vi "Knock Sensor.vi"() -> ()   [LabVIEW 2016]
doc: "This example demonstrates how to acquire a single buffer of voltage measurements using a DAQmx device.\n\nFor instructions on how to connect your signals to the DAQ device, refer to your device documentation."
uses:
  <vilib>/Utility/error.llb/DialogType.ctl
  <vilib>/DAQmx/read.llb/DAQmx Read (Analog Wfm 1Chan NSamp Duration).vi
  <vilib>/addons/_NISVFA/_Spectrum Processing/SVFA Unit Conversion (1 Ch).vi
  <vilib>/addons/_NISVFA/_Spectrum Processing/SVFA Power in Band (1 Ch).vi
  <vilib>/addons/_NISVFA/_Shared subVIs/Common/svc_Spectrum Units.vi
  <vilib>/addons/_NISVFA/_Spectrum Processing/subVIs/svfa_Conversion Utility (spectrum info).vi
  <vilib>/addons/_NISVFA/_Spectrum Processing/SVFA Get Spectrum Subset.vi
  <vilib>/addons/_NISVFA/_Spectrum Processing/SVFA Get Spectrum Subset (1 Ch).vi
  <vilib>/addons/_NISVFA/_Spectrum Processing/subVIs/svfa_Peak to RMS to Peak2Peak.vi
  <vilib>/addons/_NISVFA/_Spectrum Processing/subVIs/svfa_Mag to Mag2.vi
  <vilib>/addons/_NISVFA/_Spectrum Processing/subVIs/svfa_Linear to dB.vi
  <vilib>/addons/_NISVFA/_Spectrum Processing/subVIs/svfa_dBrefA to dBrefB.vi
  <vilib>/addons/_NISVFA/_Spectrum Processing/subVIs/svfa_Spectrum to Spectral Density.vi
  <vilib>/DAQmx/create/channels.llb/DAQmx Create Channel (AI-Voltage-Basic).vi
  <vilib>/DAQmx/configure/timing.llb/DAQmx Timing (Sample Clock).vi
  <vilib>/DAQmx/miscellaneous.llb/DAQmx Fill In Error Info.vi
  <vilib>/addons/_NISVFA/_Baseband FFT/SVFA Power Spectrum (1 Ch).vi
  <vilib>/addons/_NISVFA/_Shared subVIs/Common/svc_Format Value (DBL).vi
  <vilib>/addons/_NISVFA/_Shared subVIs/Common/svc_Engineering Units to Unit Label.vi
  <vilib>/addons/_NISVFA/_Shared subVIs/Common/svc_Unit Label Lexical Class.vi
  <vilib>/addons/_NISVFA/_Shared subVIs/Common/svc_Get Weighting Enum and Labels.vi
  <vilib>/addons/_NISVFA/_Shared subVIs/Common/svc_Window Parameters.vi
  <vilib>/addons/_NISVFA/_Shared subVIs/Common/svc_Caller VI Returned in Error Source.vi
  <vilib>/addons/_NISVFA/_Shared subVIs/Common/svc_Check Frequency Range in Spectrum.vi
  <vilib>/addons/_NISVFA/_Shared subVIs/Common/svc_Convert Frequency to Frequency String.vi
  <vilib>/addons/_NISVFA/_Shared subVIs/Common/svc_Build Unit Label for Frequency Range.vi
  <vilib>/addons/_NISVFA/_Spectrum Processing/subVIs/svfa_Spectrum Info Window to windowTd Type Def.vi
panel:
  out "All duration within tolerance":bool=TRUE
  out "Measured Knock Magnitude":dbl=5.233809983966037
  in  "RPM":dbl=6000.0
  out "Pass?":bool
  out "Measured Base Magnitude":dbl=0.1959823715521759
  out "Indice of Samples of Base Component":i32[](array[numeric])
  out "Indice of Samples of Knock Component":i32[](array[numeric])
  out "Extracted Base Spectrum":cluster{"x0":dbl, "dx":dbl, "magnitude":dbl[]}(graph)={"x0"=0.0, "dx"=0.2253587147341788, "magnitude"=array[221869 elements]}
  out "Extracted Knock Spectrum":cluster{"x0":dbl, "dx":dbl, "magnitude":dbl[]}(graph)={"x0"=0.0, "dx"=1.9895350456598349, "magnitude"=array[25132 elements]}
  out "Extracted Knock Waveform":waveform(dbl)(graph)={"t0"=timestamp(0 s since 1904-01-01), "dt"=9.999999999999972e-06, "Y"=array[50263 elements]}
  out "Extracted Base Waveform":waveform(dbl)(graph)={"t0"=timestamp(0 s since 1904-01-01), "dt"=9.999999999999972e-06, "Y"=array[443737 elements]}
  in  "Knock Duration":dbl=0.002
  in  "Knock Amplityde":dbl=5.0
  in  "Base Frequency":dbl=6500.0
  in  "Base Amplitude":dbl=0.2
  in  "Knock Frequency":dbl=2000.0
  in  "Moving Window Size(how much of one knock cycle)":dbl=0.5
  out "Waveform Graph":waveform(dbl)(graph)={"t0"=timestamp(3584720197.6212864 s since 1904-01-01), "dt"=9.999999999999972e-06, "Y"=array[500000 elements], "attributes"=variant("NI_ChannelName"=variant(string "cDAQ1Mod3/ai1"), "NI_UnitDescription"=variant(string "Volts"))}
  in  "Sampling Rate":dbl=100000.0
  in  "Duration":i32=5
  in  "Sample Clock Source":tag="OnboardClock"
  in  "Terminal Configuration":i32(ring)=-1 items=["default"=-1, "RSE"=10083, "NRSE"=10078, "Differential"=10106, "Pseudodifferential"=12529]
  in  "Max Voltage":dbl=10.0
  in  "Min Voltage":dbl=-10.0
  in  "Physical Channel":tag="cDAQ1Mod3/ai1"
  # "This test uses a moving window to separate base component and knock component from the raw signal\nand verifies the frquency and magnitude of these two components, and duration of each knock event."
  # "Channel Settings"
  # "Acquired Data"
  # "Timing Settings"
  # "Extracted Knock Component Waveform"
  # "Extracted Knock Component Spectrum"
  # "Signal Parameters"
  # "Extracted Base Component Waveform"
  # "Extracted Base Component Spectrum"
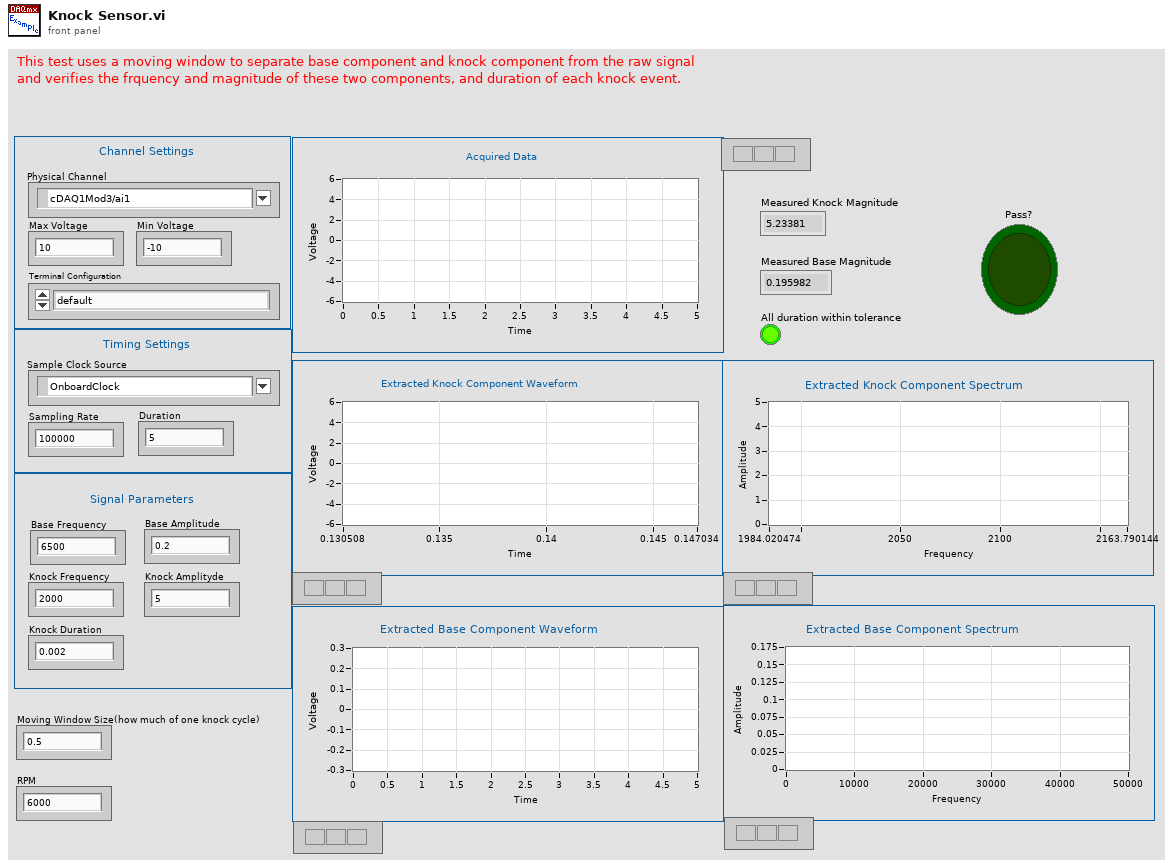
[diagram p1: front panel]
types:
  T1 = cluster{"linear/dB":enum16{"no change", "linear", "dB"}, "dB reference (0: no change)":dbl, "power/magnitude":enum16{"no change", "power", "magnitude"}, "view":enum16{"no change", "rms", "peak", "peak-peak"}}
  T2 = typedef "DialogType.ctl" = u16
  T3 = typedef "svc_Spectrum Info.ctl" = cluster{"channel name":string, "description":string, "x-axis units":T4, "spectral info":cluster{"spectrum type":T5, "linear/dB":enum16{"linear", "dB"}, "window":u16, "window size":i32, "FFT size":i32}, "engineering units":T6, "custom label":string, "dB reference [EU]":dbl, "peak units":enum16{"rms", "peak", "peak-peak"}, "weighting filter":T7, "spectral density?":bool, "unit label":string, "spectrum skewed?":bool, "complimentary spectrum units":T8}
  T4 = typedef "svc_X-Axis Units.ctl" = u16
  T5 = typedef "svc_Spectrum Type.ctl" = enum16{"FFT Spectrum [complex]", "Amplitude [Magnitude]", "Power [Magnitude^2]", "Cross Spectrum [complex]", "Frequency Response [Complex]"}
  T6 = typedef "svc_Engineering Units Text Ring.ctl" = u16
  T7 = typedef "svc_Weighting Filter Text Ring.ctl" = u16
  T8 = typedef "svc_Complimentary Spectrum Units.ctl" = enum16{"none", "radians", "degrees", "cycles", "imaginary"}
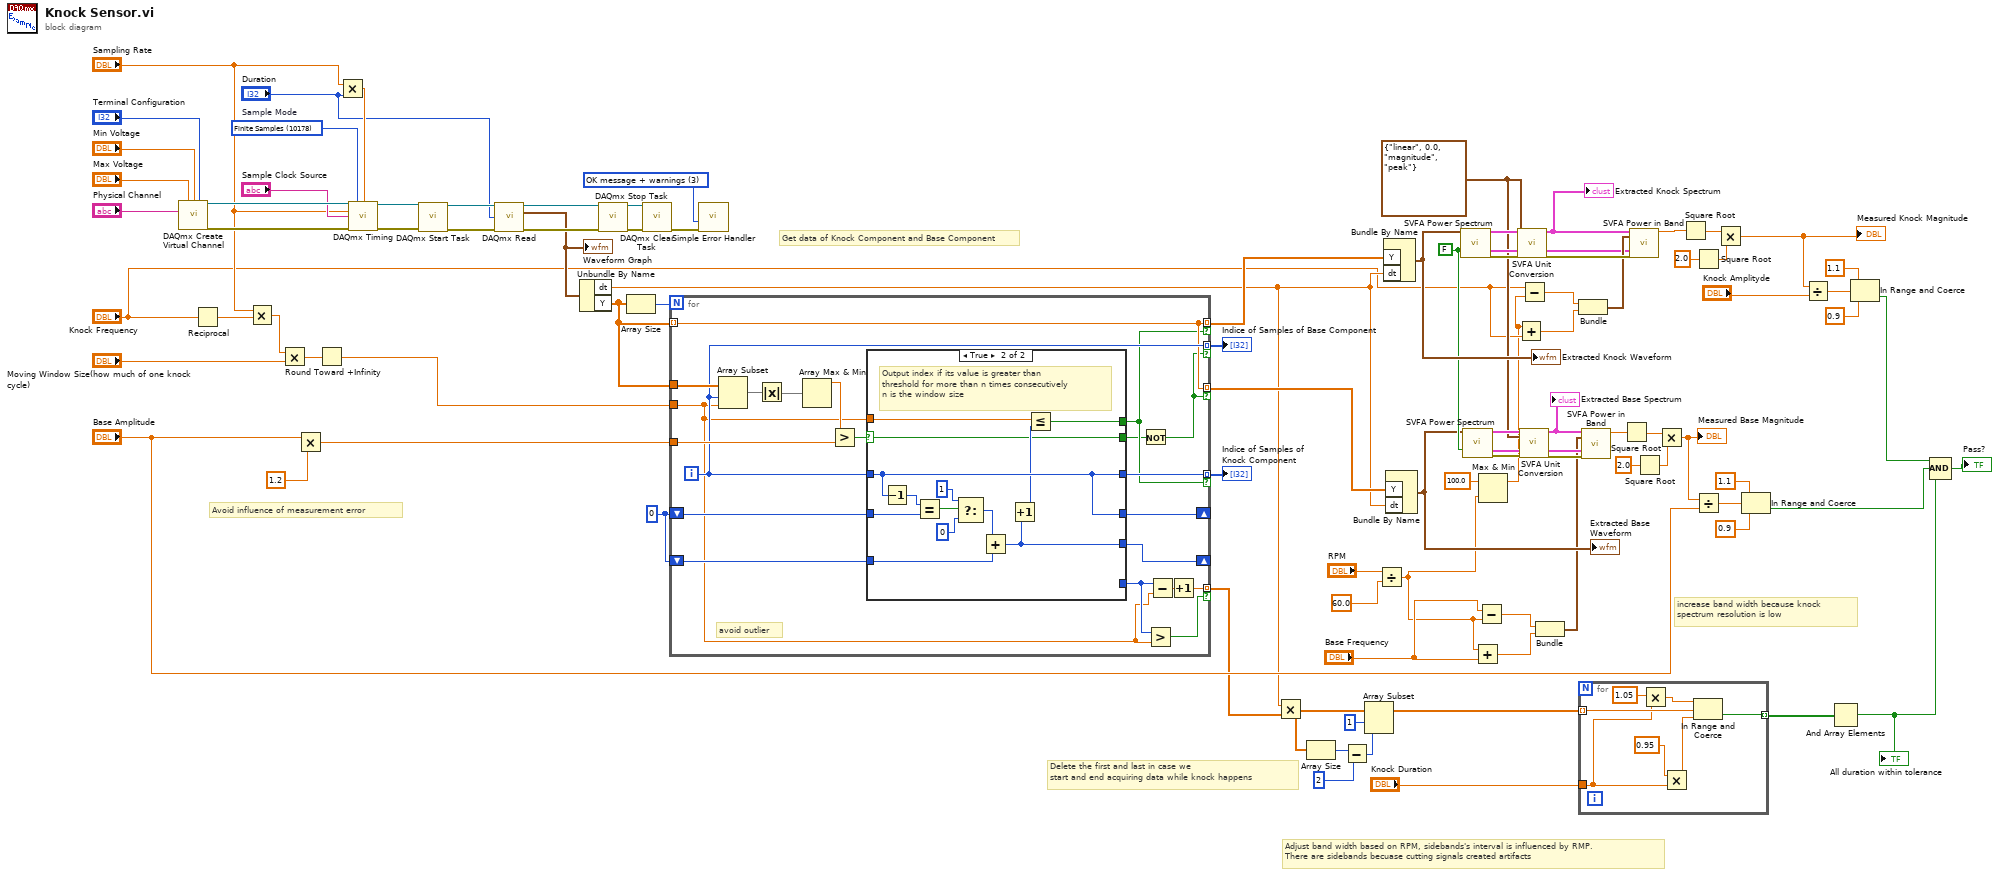
[diagram p0: block diagram]
diagram:
  w66 = 0
  w58 = T1 {"linear/dB"=enum."linear", "dB reference (0: no change)"=0.0, "power/magnitude"=enum."magnitude", "view"=enum."peak"} ("desired scaling")
  w60 = FALSE ("dB On (T)")
  w82 = T2 3 items=["no dialog", "OK message", "continue or stop message", "OK message + warnings", "continue/stop + warnings"] ("type of dialog (OK msg:1)")
  w97 = 10178 items=["Finite Samples"=10178, "Continuous Samples"=10123, "Hardware Timed Single Point"=12522]  # Sample Mode
  # "increase band width because knock \nspectrum resolution is low"
  # "Delete the first and last in case we\nstart and end acquiring data while knock happens"
  # "Adjust band width based on RPM, sidebands's interval is influenced by RMP.\nThere are sidebands becuase cutting signals created artifacts"
  # "Get data of Knock Component and Base Component"
  # "Avoid influence of measurement error"
  n1 = call-poly <vilib>:"DAQmx Create Virtual Channel.vi"("maximum value"="Max Voltage", "minimum value"="Min Voltage", "input terminal configuration"="Terminal Configuration", "physical channels"="Physical Channel") -> ("task out"=w95:refnum<k21>, "error out"=w96:errorcluster)  [unwired: 10 in]
  n2 = Reciprocal(x="Knock Frequency") -> (1/x=w77:dbl)
  n3 = Multiply(x="Sampling Rate", y=w77) -> (x*y=w75:dbl)
  n4 = Multiply(x=w75, y="Moving Window Size(how much of one knock cycle)") -> (x*y=w74:dbl)
  n5 = Multiply(x="Base Amplitude", y=1.2) -> (x*y=w40:dbl)
  n6 = Round Toward +Infinity(x=w74) -> (ceil(x): smallest int >= x=w73:dbl)
  n7 = Multiply(x="Sampling Rate", y="Duration") -> (x*y=w79:dbl)
  n8 = call-poly <vilib>:"DAQmx Timing.vi"("task/channels in"=w95, "sample mode"=w97, "samples per channel"=w79, "rate"="Sampling Rate", "source"="Sample Clock Source", "error in"=w96) -> ("task out"=w81:refnum<k21>, "error out"=w80:errorcluster)  [unwired: 8 in]
  n9 = call <vilib>:"DAQmx Start Task.vi"("task/channels in"=w81, "error in"=w80) -> ("task out"=w94:refnum<k21>, "error out"=w93:errorcluster)  [unwired: 12 in]
  n10 = call-poly <vilib>:"DAQmx Read.vi"("task/channels in"=w94, "duration"="Duration", "error in"=w93) -> ("task out"=w84:refnum<k21>, "data"=w70:waveform(dbl), "error out"=w83:errorcluster)  [unwired: 10 in]
  "Waveform Graph" <- w70
  n11 = Unbundle By Name(w70) -> ("dt"=w20:dbl, "Y"=w57:dbl[])
  n12 = call <vilib>:"DAQmx Stop Task.vi"("task/channels in"=w84, "error in"=w83) -> ("task out"=w86:refnum<k21>, "error out"=w85:errorcluster)  [unwired: 12 in]
  n13 = Array Size(array=w57) -> (size(s)=w65:i32)
  n14 = call <vilib>:"DAQmx Clear Task.vi"("task in"=w86, "error in"=w85) -> ("error out"=w92:errorcluster)  [unwired: 13 in]
  n15 = for {
    N: w65 -> [_]
    tunnel: w57 -> [w114]
    tunnel: w73 -> [w99]
    tunnel: w40 -> [w115]
    shift-right: [w111] -> _
    shift-left: w66 -> [w112]
    shift-right: [w103] -> _
    shift-left: w66 -> [w110]
    tunnel: [w109] -> w56 mode=indexing if=w106
    tunnel: [w108] -> w55 mode=indexing if=w104
    tunnel: w57 -> [w107] mode=indexing
    tunnel: [w107] -> w32 mode=indexing if=w106
    tunnel: [w107] -> w54 mode=indexing if=w104
    tunnel: [w98] -> w31 mode=indexing if=w102
    i -> [w108]
    # "avoid outlier"
    n16 = Array Subset(array=w114, index=w108, length=w99) -> (w118:dbl[])
    n17 = Absolute Value(x=w118) -> (abs(x)=w117:dbl[])
    n18 = Array Max & Min(array=w117) -> (max value=w116:dbl)  [unwired: 3 out]
    n19 = Greater?(x=w116, y=w115) -> (0:w113:bool)
    n20 = case shown="True" w113 {
      selector: w113 -> [w120 w122]
      tunnel: w108 -> [_ w125]
      tunnel: w112 -> [w121 w133]
      tunnel: [w121 w125] -> w111
      tunnel: w110 -> [w119 w128]
      tunnel: w99 -> [_ w123]
      tunnel: [_ w127] -> w103
      tunnel: [_ w125] -> w109
      tunnel: [_ w126] -> w106
      tunnel: [w120 w122] -> w105
      tunnel: [w119 _] -> w100
      frame False {
      }
      frame True {
        # "Output index if its value is greater than \nthreshold for more than n times consecutively\nn is the window size"
        n21 = Decrement(x=w125) -> (x-1=w134:i32)
        n22 = Equal?(x=w134, y=w133) -> (x = y?=w132:bool)
        n23 = Select(t=1, s=w132, f=0) -> (s? t:f=w129:i32)
        n24 = Add(x=w129, y=w128) -> (x+y=w127:i32)
        n25 = Increment(x=w127) -> (x+1=w124:i32)
        n26 = Less Or Equal?(x=w123, y=w124) -> (x <= y?=w126:bool)
      }
    }
    n27 = Not(x=w105) -> (.not. x?=w104:bool)
    n28 = Greater?(x=w100, y=w99) -> (0:w102:bool)
    n29 = Subtract(x=w100, y=w99) -> (x-y=w101:dbl)
    n30 = Increment(x=w101) -> (x+1=w98:dbl)
  }
  "Indice of Samples of Knock Component" <- w56
  "Indice of Samples of Base Component" <- w55
  n31 = call <vilib>:"Simple Error Handler.vi"("type of dialog (OK msg:1)"=w82, "error in (no error)"=w92) -> ()  [unwired: 3 in, 5 out]
  n32 = Multiply(x=w20, y=w31) -> (x*y=w10:dbl[])
  n33 = Array Size(array=w10) -> (size(s)=w9:i32)
  n34 = Subtract(x=w9, y=2) -> (x-y=w7:i32)
  n35 = Array Subset(array=w10, index=1, length=w7) -> (w12:dbl[])
  n36 = Divide(x="RPM", y=60.0) -> (x/y=w1:dbl)
  n37 = Bundle By Name("Y"=w32, "dt"=w20) -> (w64:waveform(dbl))  [unwired: 1 in]
  "Extracted Knock Waveform" <- w64
  n38 = Bundle By Name("Y"=w54, "dt"=w20) -> (w59:waveform(dbl))  [unwired: 1 in]
  "Extracted Base Waveform" <- w59
  n39 = call-poly <vilib>:"SVFA Power Spectrum.vi"("scaled signal [EU]"=w64, "dB On (T)"=w60) -> ("power spectrum [dB EU]"=w67:cluster{"f0":dbl, "df":dbl, "magnitude":dbl[]}, "spectrum info"=w68:T3, "error out"=w69:errorcluster)  [unwired: 12 in, 3 out]
  n40 = call-poly <vilib>:"SVFA Power Spectrum.vi"("scaled signal [EU]"=w59, "dB On (T)"=w60) -> ("power spectrum [dB EU]"=w63:cluster{"f0":dbl, "df":dbl, "magnitude":dbl[]}, "spectrum info"=w62:T3, "error out"=w61:errorcluster)  [unwired: 12 in, 3 out]
  n41 = Add(x=w1, y="Base Frequency") -> (x+y=w53:dbl)
  n42 = Subtract(x="Base Frequency", y=w1) -> (x-y=w52:dbl)
  n43 = Max & Min(x=100.0, y=w1) -> (max(x,y)=w3:dbl)  [unwired: 1 out]
  n44 = Add(x=w3, y="Knock Frequency") -> (x+y=w21:dbl)
  n45 = call-poly <vilib>:"SVFA Unit Conversion.vi"("spectrum"=w67, "desired scaling"=w58, "spectrum info in"=w68, "error in (no error)"=w69) -> ("converted spectrum"=w6:cluster{"x0":dbl, "dx":dbl, "magnitude":dbl[]}, "spectrum info out"=w5:T3, "error out"=w23:errorcluster)  [unwired: 12 in, 1 out]
  "Extracted Knock Spectrum" <- w6
  n46 = call-poly <vilib>:"SVFA Unit Conversion.vi"("spectrum"=w63, "desired scaling"=w58, "spectrum info in"=w62, "error in (no error)"=w61) -> ("converted spectrum"=w49:cluster{"x0":dbl, "dx":dbl, "magnitude":dbl[]}, "spectrum info out"=w51:T3, "error out"=w50:errorcluster)  [unwired: 12 in, 1 out]
  "Extracted Base Spectrum" <- w49
  n47 = Subtract(x="Knock Frequency", y=w3) -> (x-y=w22:dbl)
  n48 = Bundle(w52, w53) -> (w48:cluster{dbl, dbl})  [unwired: 1 in]
  n49 = Bundle(w22, w21) -> (w18:cluster{dbl, dbl})  [unwired: 1 in]
  n50 = for {
    tunnel: w12 -> [w141] mode=indexing
    tunnel: "Knock Duration" -> [w138]
    tunnel: [w136] -> w29 mode=indexing
    n51 = Multiply(x=1.05 ("upper limit"), y=w138) -> (x*y=w139:dbl)
    n52 = Multiply(x=0.95 ("lower limit"), y=w138) -> (x*y=w135:dbl)
    n53 = In Range and Coerce(upper limit=w139, x=w141, lower limit=w135) -> (In Range?=w136:bool)  [unwired: 1 out]
  }
  n54 = call-poly <vilib>:"SVFA Power in Band.vi"("spectrum"=w49, "range"=w48, "spectrum info"=w51, "error in (no error)"=w50) -> ("power in band"=w43:dbl)  [unwired: 13 in, 2 out]
  n55 = Square Root(x=w43) -> (sqrt(x)=w44:dbl)
  n56 = call-poly <vilib>:"SVFA Power in Band.vi"("spectrum"=w6, "range"=w18, "spectrum info"=w5, "error in (no error)"=w23) -> ("power in band"=w14:dbl)  [unwired: 13 in, 2 out]
  n57 = Square Root(x=2.0) -> (sqrt(x)=w45:dbl)
  n58 = Multiply(x=w44, y=w45) -> (x*y=w42:dbl)
  "Measured Base Magnitude" <- w42
  n59 = Square Root(x=w14) -> (sqrt(x)=w17:dbl)
  n60 = Square Root(x=2.0) -> (sqrt(x)=w16:dbl)
  n61 = Divide(x=w42, y="Base Amplitude") -> (x/y=w39:dbl)
  n62 = Multiply(x=w17, y=w16) -> (x*y=w13:dbl)
  "Measured Knock Magnitude" <- w13
  n63 = In Range and Coerce(upper limit=1.1, x=w39, lower limit=0.9) -> (In Range?=w28:bool)  [unwired: 1 out]
  n64 = Divide(x=w13, y="Knock Amplityde") -> (x/y=w34:dbl)
  n65 = And Array Elements(Boolean array=w29) -> (logical AND=w27:bool)
  "All duration within tolerance" <- w27
  n66 = In Range and Coerce(upper limit=1.1, x=w34, lower limit=0.9) -> (In Range?=w4:bool)  [unwired: 1 out]
  n67 = Compound Arithmetic op=AND(w4, w28, w27) -> (→"Pass?":bool)
